vi "Get driving mode to excecute.vi"() -> (0 "Drive Mode":T1=enum."Driver Operated")   [LabVIEW 2018]
uses:
  Drive mode.ctl
  Robot Global Data.vi
  <vilib>/Rock Robotics/Network Tables/NT Read Boolean.vi
panel:
  # "Choose which mode to excecute"
  # "IDK HOw this is going to work exactly"
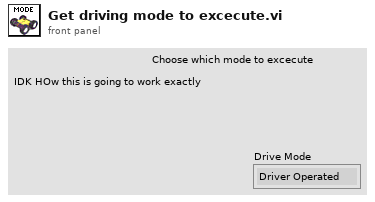
[diagram p1: front panel]
types:
  T1 = typedef "Drive mode.ctl" = enum16{"HAB2toHAB1", "Driver Operated", "Drive Autonomously", "Disabled"}
  T2 = typedef "WPI_DriverStationRobotMode2.ctl" = enum16{"Autonomous Disabled", "Autonomous Enabled", "Teleop Disabled", "Teleop Enabled", "Disconnected", "Finish", "Test Disabled", "Test Enabled", "Emergency Stopped"}
  T3 = cluster{"Left Motor Value":dbl, "Right Motor Value":dbl}
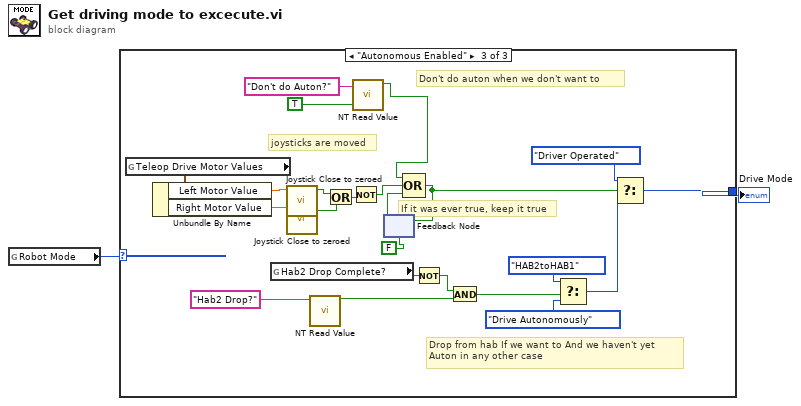
[diagram p0: block diagram]
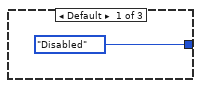
[diagram p2: hidden frame]
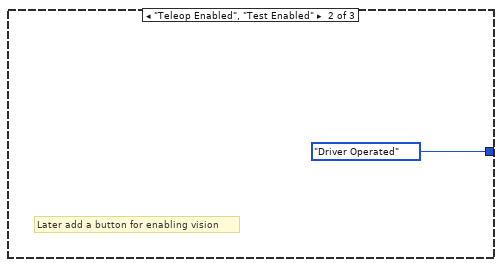
[diagram p3: hidden frame]
diagram:
  n1 = global read "Robot Global Data.vi" "Robot Mode"() -> (w2:T2)
  n2 = case shown="\"Autonomous Enabled\"" w2 {
    tunnel: [Drive_mode."Disabled" ("Drive Mode") Drive_mode."Driver Operated" ("Drive Mode") w22] -> w1
    frame Default {
    }
    frame "Teleop Enabled", "Test Enabled" {
      # "Later add a button for enabling vision"
    }
    frame "Autonomous Enabled" {
      # "Don't do auton when we don't want to"
      # "Drop from hab If we want to And we haven't yet\nAuton in any other case"
      # "joysticks are moved"
      # "If it was ever true, keep it true"
      n3 = global read "Robot Global Data.vi" "Teleop Drive Motor Values"() -> (w23:T3)
      n4 = Unbundle By Name(w23) -> ("Left Motor Value"=w24:dbl, "Right Motor Value"=w25:dbl)
      n5 = global read "Robot Global Data.vi" "Hab2 Drop Complete?"() -> (w11:bool)
      n6 = call "Joystick Close to zeroed.vi"("Joystick"=w24) -> ("=0?"=w27:bool)  [unwired: 10 in]
      n7 = call "Joystick Close to zeroed.vi"("Joystick"=w25) -> ("=0?"=w26:bool)  [unwired: 10 in]
      n8 = call-poly <vilib>:"NT Read Value.vi"("Name"="Hab2 Drop?") -> ("Boolean"=w13:bool)  [unwired: 9 in, 1 out]
      n9 = Or(x=w27, y=w26) -> (x .or. y?=w15:bool)
      n10 = Not(x=w15) -> (.not. x?=w9:bool)
      n11 = call-poly <vilib>:"NT Read Value.vi"("Default Value"=TRUE, "Name"="Don't do Auton?") -> ("Boolean"=w5:bool)  [unwired: 8 in, 1 out]
      n12 = feedback #1(FALSE) -> (w10:bool)
      n13 = Compound Arithmetic op=OR(w5, w9, w10) -> (w7:bool)
      n14 = feedback-in #1(w7) -> ()
      n15 = Not(x=w11) -> (.not. x?=w12:bool)
      n16 = And(x=w12, y=w13) -> (x .and. y?=w14:bool)
      n17 = Select(t=Drive_mode."HAB2toHAB1" ("Drive Mode"), s=w14, f=Drive_mode."Drive Autonomously" ("Drive Mode")) -> (s? t:f=w18:T1)
      n18 = Select(t=Drive_mode."Driver Operated" ("Drive Mode"), s=w7, f=w18) -> (s? t:f=w22:T1)
    }
  }
  "Drive Mode" <- w1
